vi "Set Parameters File MD5 Checksum.vi"(8 "error in":errorcluster, 9 "MD5":string, 11 "custom device ref":T1 format="%.0x") -> (0 "error out":errorcluster, 3 "custom device ref out":T1 format="%.0x")   [LabVIEW 2020, in "Ballard ARINC 429 Scripting.lvlib"]
uses:
  Ballard ARINC 429 Scripting.lvlib
  <vilib>/NI VeriStand/Custom Device API/Custom Device API.lvlib
  Constants.vi
  <vilib>/NI VeriStand/Custom Device API/Set Item Property (String).vi
  <vilib>/NI VeriStand/Custom Device API/Custom Device Item Ref.ctl
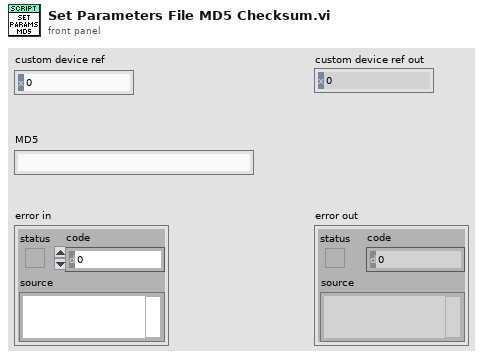
[diagram p1: front panel]
types:
  T1 = typedef "Custom Device API.lvlib/Custom Device Item Ref.ctl" = u64
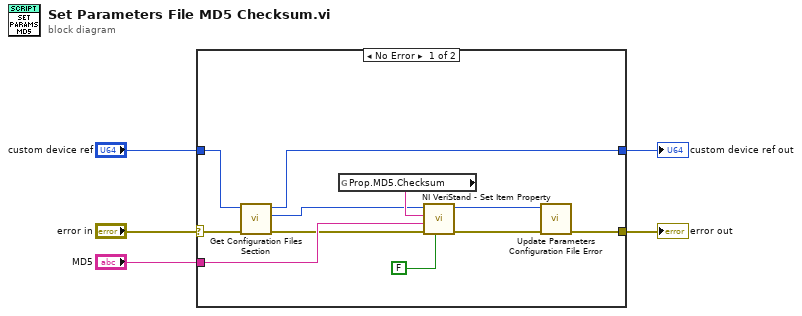
[diagram p0: block diagram]
diagram:
  n1 = case shown="No Error" "error in" {
    selector: "error in" -> [w11 w18]
    tunnel: "custom device ref" -> [w8 w17]
    tunnel: [w12 w18] -> w4
    tunnel: "MD5" -> [w16 _]
    tunnel: [w7 w17] -> w1
    frame No Error {
      n2 = call "Get Configuration Files Section.vi"("error in"=w11, "Custom device Ref"=w8) -> ("error out"=w10:errorcluster, "Configuration files Ref"=w9:T1, "Custom device Ref out"=w7:T1)  [unwired: 7 in]
      n3 = global read "Constants.vi" "Prop.MD5.Checksum"() -> (w15:string)
      n4 = call-poly <vilib>:"NI VeriStand - Set Item Property.vi"("Binary String (T)"=FALSE, "error in (no error)"=w10, "Value"=w16, "Property Name"=w15, "Item Ref in"=w9) -> ("error out"=w13:errorcluster, "Item Ref out"=w14:T1)  [unwired: 4 in, 1 out]
      n5 = call "Update Parameters Configuration File Error.vi"("error in"=w13, "Configuration files Ref"=w14) -> ("error out"=w12:errorcluster)  [unwired: 8 in, 1 out]
    }
    frame Error {
    }
  }
  "error out" <- w4
  "custom device ref out" <- w1
